vi "onTestExecution.vi"(6 "timeout (2000 ms)":i32=2000, 7 "Name":string, 8 "error in (no error)":errorcluster, 11 "Test Runner.Project in":refnum<class "Test Runner.Class.lvclass">) -> (0 "error out":errorcluster, 3 "Test Runner.Project out":refnum<class "Test Runner.Class.lvclass">)   [LabVIEW 2020, in "Caraya.lvlib" / "Test Runner.Class.lvclass"]
uses:
  Test Runner.Class.lvclass
  C:/projects/caraya/src/classes/Test Runner/Test Runner.lvclass
  Test Runner.Class.lvclass/Test Runner.Class.ctl
  Assert/Assert True.vi
  Assert/Assert.lvclass
  Test Runner/Test Runner.lvclass
  Test/Test.lvclass
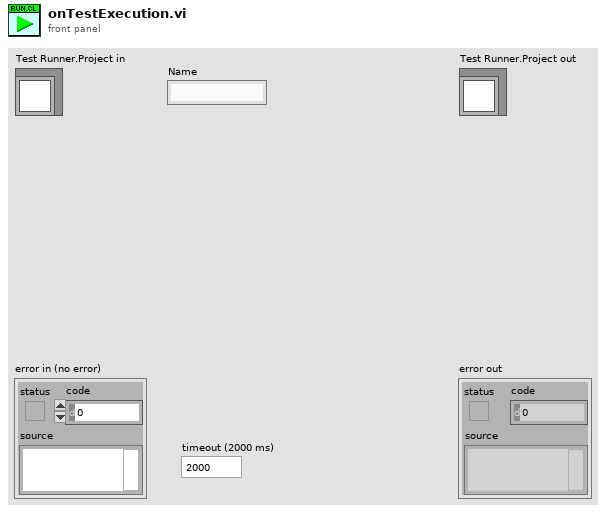
[diagram p1: front panel]
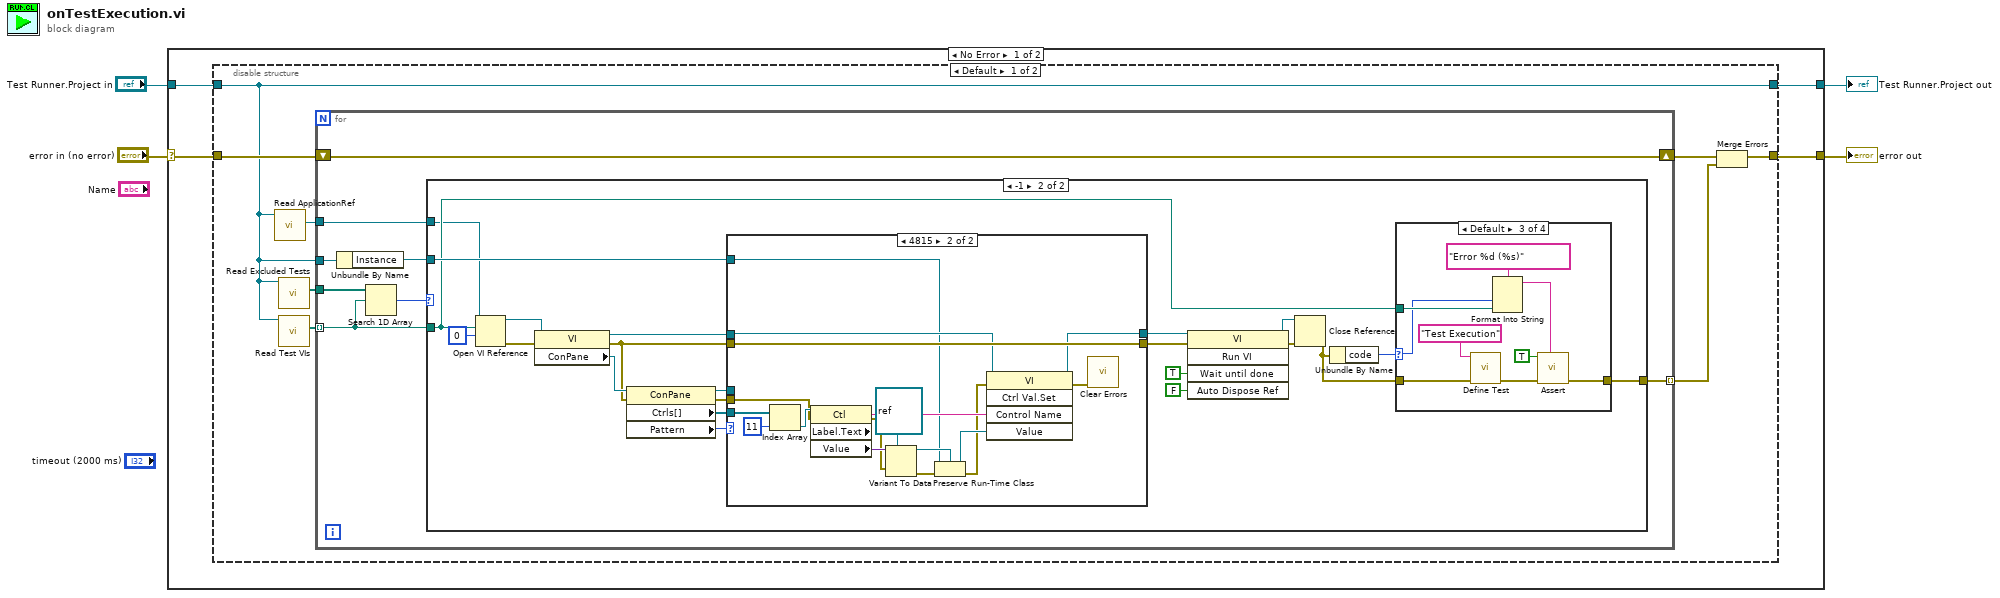
[diagram p0: block diagram]
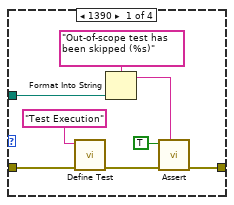
[diagram p4: hidden frame]
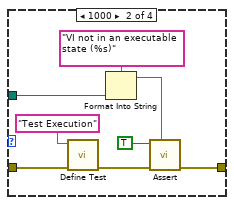
[diagram p5: hidden frame]
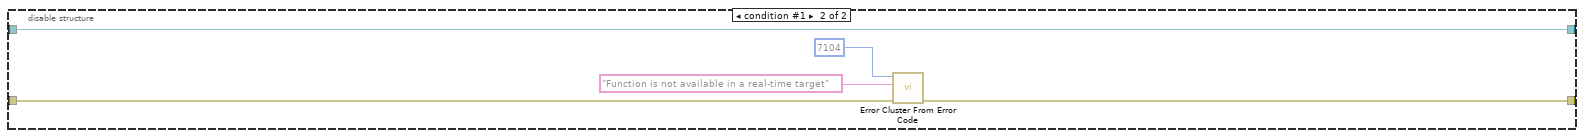
[diagram p7: hidden frame]
diagram:
  n1 = case shown="No Error" "error in (no error)" {
    selector: "error in (no error)" -> [w8 w98]
    tunnel: "Test Runner.Project in" -> [w7 w97]
    tunnel: [w6 w97] -> w4
    tunnel: [w5 w98] -> w3
    frame No Error {
      n2 = disable-structure shown="Default" {
        disable-tunnel: w8 -> [w11 w93]
        disable-tunnel: [w12 w92] -> w5
        disable-tunnel: w7 -> [w10 w96]
        disable-tunnel: [w10 w96] -> w6
        frame condition #0 (active) {
          n3 = call "Read ApplicationRef.vi"("Test Runner in"=w10) -> ("Application"=w9:refnum<vi>)  [unwired: 8 in, 2 out]
          n4 = call "Read Excluded Tests.vi"("Test Runner in"=w10) -> ("Excluded Tests"=w15:path[])  [unwired: 8 in, 2 out]
          n5 = call "Read Test VIs.vi"("Test Runner in"=w10) -> ("Test VIs"=w14:path[])  [unwired: 8 in, 2 out]
          n6 = for {
            tunnel: w14 -> [w23] mode=indexing
            tunnel: [w22] -> w16 mode=indexing
            tunnel: w15 -> [w24]
            shift-right: [w20] -> w13
            shift-left: w11 -> [w20]
            tunnel: w10 -> [w19]
            tunnel: w9 -> [w17]
            n7 = Unbundle By Name(w19) -> ("Instance"=w18:refnum<class>)
            n8 = Search 1D Array(1D array=w24, element=w23) -> (index of element=w21:i32)  [unwired: 1 in]
            n9 = case shown="-1" w21 {
              tunnel: w23 -> [_ w27]
              tunnel: [_ w40] -> w22
              tunnel: w18 -> [_ w33]
              tunnel: w17 -> [_ w25]
              frame Default {
                # "Test is part of the exclusion list"
              }
              frame -1 {
                n10 = Open VI Reference(application reference (local)=w25, vi path=w27, options=0) -> (vi reference=w26:refnum<vi>, error out=w39:errorcluster)  [unwired: 3 in]
                n11 = property class="VI"(reference=w26, error in=w39) -> (reference out=w32:refnum<vi>, error out=w30:errorcluster, "ConPane"=w36:refnum<vi>)
                n12 = property class="ConPane"(reference=w36, error in=w30) -> (reference out=w35:refnum<vi>, error out=w34:errorcluster, "Ctrls[]"=w38:refnum<vi>[], "Pattern"=w37:u32)
                n13 = case shown="4815" w37 {
                  tunnel: w38 -> [_ w65]
                  tunnel: w35 -> [_ _]
                  tunnel: w34 -> [_ w59]
                  tunnel: w33 -> [_ w50]
                  tunnel: w32 -> [w48 w55]
                  tunnel: [w48 w54] -> w31
                  tunnel: w30 -> [w47 w57]
                  tunnel: [w47 w57] -> w29
                  frame 0, Default {
                  }
                  frame 4815 {
                    n14 = Index Array(array=w65, index=11) -> (element=w63:refnum<vi>)
                    n15 = property class="Ctl"(reference=w63, error in=w59) -> (error out=w58:errorcluster, "Label.Text"=w52:string, "Value"=w62:variant)  [unwired: 1 out]
                    n16 = Variant To Data(error in=w58, type=refnum<class> refnum ("Instance"), Variant=w62) -> (data=w51:refnum<class>, error out=w60:errorcluster)
                    n17 = Preserve Run-Time Class(object in=w50, error in=w60, 2:w51) -> (object out=w53:refnum<class>, error out=w49:errorcluster)
                    n18 = invoke on="Invoke Node" class="VI" method="Ctrl Val.Set"(reference=w55, error in=w49, "Control Name"=w52, "Value"=w53) -> (reference out=w54:refnum<vi>, error out=w56:errorcluster)  [unwired: 1 in, 3 out]
                    n19 = call <vilib>:"Clear Errors.vi"("error in (no error)"=w56) -> ()  [unwired: 5 in, 2 out]
                  }
                }
                n20 = invoke on="Invoke Node" class="VI" method="Run VI"(reference=w31, error in=w29, "Wait until done"=TRUE ("Wait Until Done"), "Auto Dispose Ref"=FALSE ("Auto Dispose Reference")) -> (reference out=w43:refnum<vi>, error out=w42:errorcluster)  [unwired: 1 in, 3 out]
                n21 = Close Reference(reference=w43, error in (no error)=w42) -> (error out=w41:errorcluster)
                n22 = Unbundle By Name(w41) -> ("code"=w44:i32)
                n23 = case shown="Default" w44 {
                  selector: w44 -> [_ _ w88 _]
                  tunnel: w41 -> [w70 w78 w86 w91]
                  tunnel: [w68 w76 w82 w91] -> w40
                  tunnel: w27 -> [w73 w81 w90 _]
                  frame 1390 {
                    n24 = call "Define Test.vi"("error in (no error)"=w70, "Label (VI Title)"="Test Execution") -> ("error out"=w69:errorcluster)  [unwired: 8 in, 1 out]
                    n25 = Format Into String(format string="Out-of-scope test has been skipped (%s)" ("Label"), w73) -> (resulting string=w67:string)  [unwired: 2 in, 1 out]
                    n26 = call-poly "Assert.vi"("Label"=w67, "error in (no error)"=w69, "True?"=TRUE) -> ("error out"=w68:errorcluster)  [unwired: 7 in, 1 out]
                  }
                  frame 1000 {
                    n27 = call "Define Test.vi"("error in (no error)"=w78, "Label (VI Title)"="Test Execution") -> ("error out"=w77:errorcluster)  [unwired: 8 in, 1 out]
                    n28 = Format Into String(format string="VI not in an executable state (%s)" ("Label"), w81) -> (resulting string=w74:string)  [unwired: 2 in, 1 out]
                    n29 = call-poly "Assert.vi"("Label"=w74, "error in (no error)"=w77, "True?"=TRUE) -> ("error out"=w76:errorcluster)  [unwired: 7 in, 1 out]
                  }
                  frame Default {
                    n30 = call "Define Test.vi"("error in (no error)"=w86, "Label (VI Title)"="Test Execution") -> ("error out"=w83:errorcluster)  [unwired: 8 in, 1 out]
                    n31 = Format Into String(format string="Error %d (%s)" ("Label"), w88, w90) -> (resulting string=w85:string)  [unwired: 2 in, 1 out]
                    n32 = call-poly "Assert.vi"("Label"=w85, "error in (no error)"=w83, "True?"=TRUE) -> ("error out"=w82:errorcluster)  [unwired: 7 in, 1 out]
                  }
                  frame 0 {
                  }
                }
              }
            }
          }
          n33 = Merge Errors(w13, w16) -> (w12:errorcluster)
        }
        frame condition #1 {
          n34 = call <vilib>:"Error Cluster From Error Code.vi"("error in (no error)"=w93, "error message (\"\")"="Function is not available in a real-time target" ("error message (\"\")"), "error code (0)"=7104) -> ("error out"=w92:errorcluster)  [unwired: 6 in]
        }
      }
    }
    frame Error {
    }
  }
  "error out" <- w3
  "Test Runner.Project out" <- w4
